vi "AddParamChannels.vi"(6 "Type":T3, 8 "error in":errorcluster, 9 "Initial Value":u32, 10 "Parameters to add":T2[](array[typedef]), 11 "Node Ref In":T1=18446744073709551615 format="%.0x") -> (0 "error out":errorcluster, 3 "Node Ref Out":T1=18446744073709551615 format="%.0x")   [LabVIEW 2015, in "AIT 429 System Explorer.lvlib"]
uses:
  AIT 429 System Explorer.lvlib
  <vilib>/NI Veristand/Custom Device API/Custom Device Item Ref.ctl
  <vilib>/NI Veristand/Custom Device API/Custom Device Channel Type.ctl
  Controls/ARINCParam.ctl
  <vilib>/NI Veristand/Custom Device API/Custom Device Channel.ctl
  Shared/Controls and Global/Global.vi
  Shared/AIT 429 Shared.lvlib
  <vilib>/NI Veristand/Custom Device API/Custom Device API.lvlib
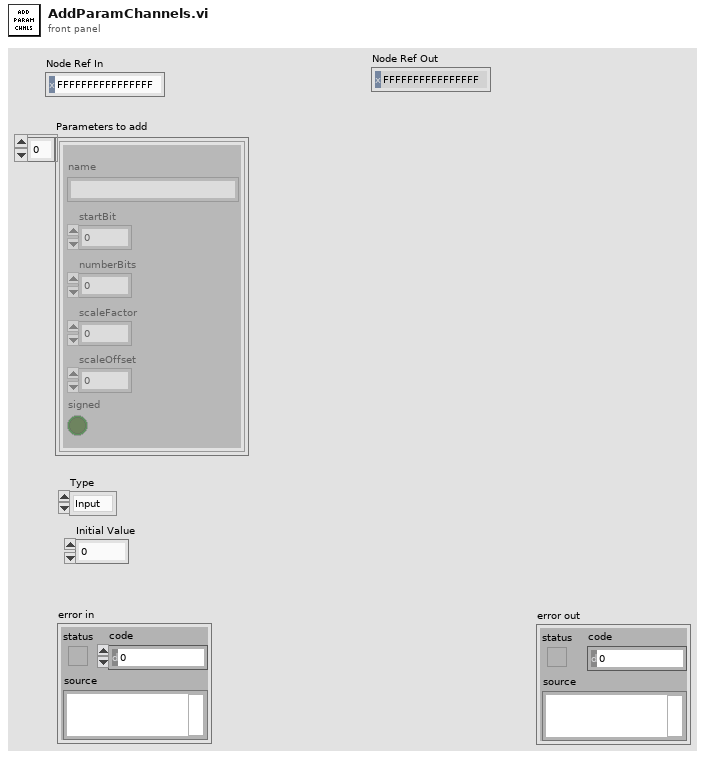
[diagram p1: front panel]
types:
  T1 = typedef "Custom Device API.lvlib/Custom Device Item Ref.ctl" = u64
  T2 = typedef "AIT 429 System Explorer.lvlib/ARINCParam.ctl" = cluster{"name":string, "startBit":i32, "numberBits":i32, "scaleFactor":dbl, "scaleOffset":dbl, "signed":bool}
  T3 = typedef "Custom Device API.lvlib/Custom Device Channel Type.ctl" = enum16{"Input", "Output"}
  T4 = typedef "Custom Device API.lvlib/Custom Device Channel.ctl" = cluster{"Type":T3, "Units":string, "Default Value":dbl, "Faultable":bool, "Scalable":bool}
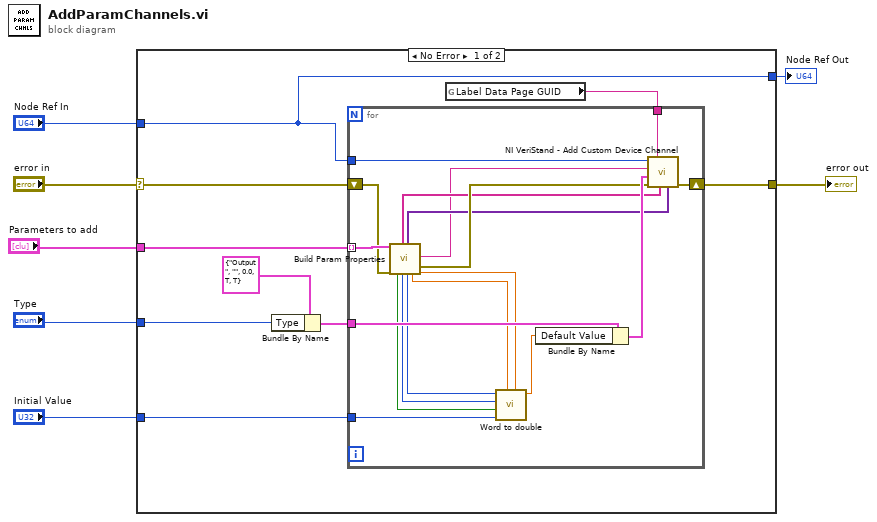
[diagram p0: block diagram]
diagram:
  n1 = case shown="No Error" "error in" {
    selector: "error in" -> [w9 w36]
    tunnel: "Parameters to add" -> [w13 _]
    tunnel: "Node Ref In" -> [w8 w35]
    tunnel: "Initial Value" -> [w12 _]
    tunnel: "Type" -> [w11 _]
    tunnel: [w10 w36] -> w4
    tunnel: [w8 w35] -> w1
    frame No Error {
      n2 = Bundle By Name(cluster=T4 {"Type"=enum."Output", "Units"="", "Default Value"=0.0, "Faultable"=TRUE, "Scalable"=TRUE} ("Channel"), "Type"=w11) -> (w15:T4)
      n3 = global read "Global.vi" "Label Data Page GUID"() -> (w16:string)
      n4 = for {
        shift-right: [w18] -> w10
        shift-left: w9 -> [w28]
        tunnel: w8 -> [w34]
        tunnel: w15 -> [w32]
        tunnel: w16 -> [w33]
        tunnel: w13 -> [w29] mode=indexing
        tunnel: w12 -> [w30]
        n5 = call "Build Param Properties.vi"("ARINC Parameter"=w29, "error in (no error)"=w28) -> ("signed"=w23:bool, "Prop Names"=w26:string[], "numberBits"=w22:i32, "Prop Values"=w25:variant[], "startBit"=w21:i32, "scaleFactor"=w20:dbl, "name"=w17:string, "error out"=w27:errorcluster, "scaleOffset"=w19:dbl)  [unwired: 9 in]
        n6 = call "Word to double.vi"("ScaleOffset (0)"=w19, "ScaleFac (1)"=w20, "word"=w30, "Signed? (F)"=w23, "Number of Bits"=w22, "Start Bit"=w21) -> ("Double"=w24:dbl)  [unwired: 5 in]
        n7 = Bundle By Name(cluster=w32, "Default Value"=w24) -> (w31:T4)
        n8 = call <vilib>:"NI VeriStand - Add Custom Device Channel.vi"("Property Values"=w25, "Property names"=w26, "GUID (Default Channel)"=w33, "error in (no error)"=w27, "Channel"=w31, "Channel Name"=w17, "Parent Ref in"=w34) -> ("error out"=w18:errorcluster)  [unwired: 1 in, 3 out]
      }
    }
    frame Error {
    }
  }
  "error out" <- w4
  "Node Ref Out" <- w1
